vi "Log Warning.vi"(8 "error in (no error)":errorcluster, 10 "Message":string, 11 "Logging In":refnum<class "Logging.lvclass">) -> (0 "error out":errorcluster, 3 "Logging Out":refnum<class "Logging.lvclass">)   [LabVIEW 2020, in "Logging.lvclass"]
doc: "Enter a warning-level message into the system log.\nA warning is an indication that something unexpected happened, or indicative of some problem in the near future (e.g. ‘disk space low’). The software is still working as expected."
uses:
  Logging.lvclass
  Protected/Level.ctl
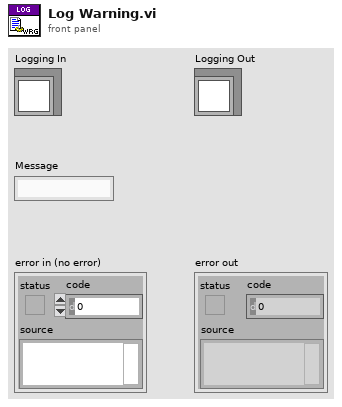
[diagram p1: front panel]
types:
  T1 = typedef "Logging.lvclass/Level.ctl" = enum16{"DEBUG", "INFO", "WARNING", "ERROR", "CRITICAL"}
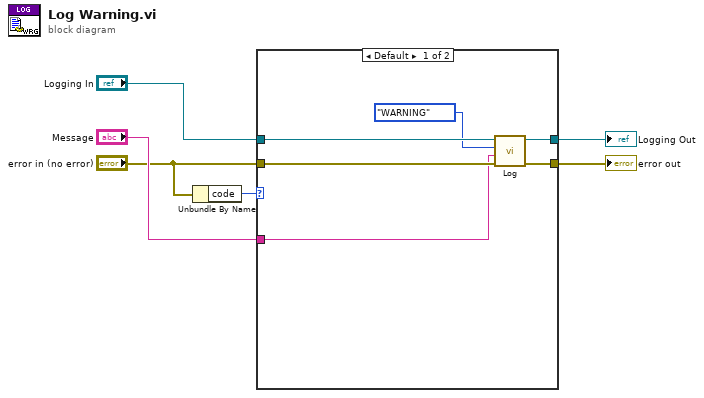
[diagram p0: block diagram]
diagram:
  n1 = Unbundle By Name("error in (no error)") -> ("code"=w1:i32)
  n2 = case shown="Default" w1 {
    tunnel: [w12 w13] -> w6
    tunnel: "Logging In" -> [w11 w14]
    tunnel: [w10 w14] -> w4
    tunnel: "Message" -> [w7 _]
    tunnel: "error in (no error)" -> [w9 w13]
    frame Default {
      n3 = call-dynamic "Log.vi"("error in (no error)"=w9, "Message"=w7, "Level"=Level."WARNING", "Logging In"=w11) -> ("error out"=w12:errorcluster, "Logging Out"=w10:refnum<class "Logging.lvclass">)  [unwired: 6 in]
    }
    frame 0 {
    }
  }
  "error out" <- w6
  "Logging Out" <- w4
